vi "PathPlanner_PathFinding_SetGoalPosition.vi"(8 "error in (no error)":errorcluster, 11 "GoalPosition":T1 {"Y" format="%14.3f"; "X" format="%14.3f"}) -> (0 "error out":errorcluster)   [LabVIEW 2019, in "PathPlanner24.lvlib"]
doc: "DOCUMENTATION NOT COMPLETE YET."
uses:
  PathPlanner24.lvlib
  <vilib>/Rock Robotics/WPI/ThirdParty/JAS_Junk/TrajLib/TypeDef/TRANSLATION2D.ctl
  ENum/PathPlanner_PathFinding_Cmd_ENUM.ctl
  <vilib>/Rock Robotics/WPI/ThirdParty/JAS_Junk/TrajLib/Translation2d_GetXY.vi
  PathPlanner_GridPosition_New.vi
  PathPlanner_GridPosition_HashCode.vi
  PathPlanner_PathFinder_GetAllNeighbors.vi
  PathPlanner_GridPosition_Get.vi
  PathPlanner_PathFinder_Globals.vi
  <vilib>/Rock Robotics/WPI/ThirdParty/JAS_Junk/TrajLib/Trajectory_Library.lvlib
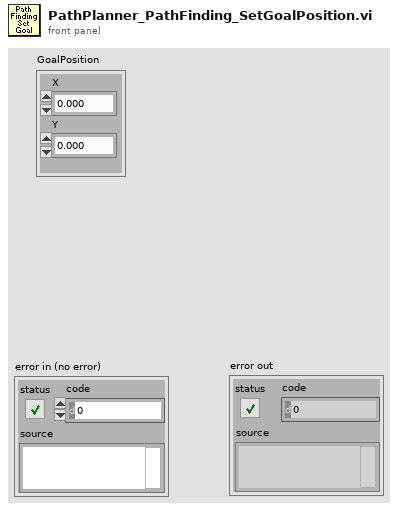
[diagram p1: front panel]
types:
  T1 = typedef "Trajectory_Library.lvlib/TRANSLATION2D.ctl" = cluster{"X":dbl, "Y":dbl}
  T2 = typedef "PathPlanner24.lvlib/PathPlannerFinderGridPosition.ctl" = cluster{"X":i32, "Y":i32}
  T3 = typedef "PathPlanner24.lvlib/PathPlanner_PathFinding_Cmd_ENUM.ctl" = enum16{"Do Nothing", "Reset", "Minor", "Reset and Minor", "Major", "Reset and Major", "Minor and Major", "Reset, Minor, Major"}
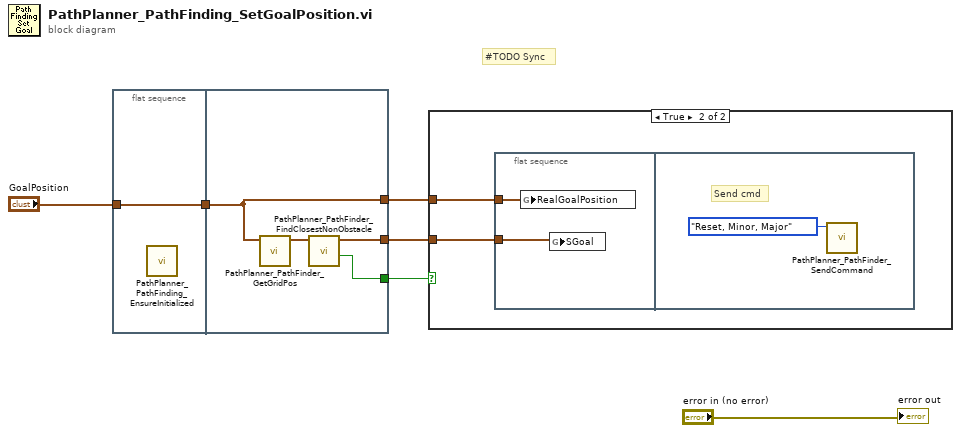
[diagram p0: block diagram]
diagram:
  # "#TODO Sync"
  n1 = flat-sequence {
    tunnel: "GoalPosition" -> [w7]
    tunnel: [w7] -> w2
    tunnel: [w10] -> w6
    tunnel: [w9] -> w5
    tunnel: w2 -> [w8]
    tunnel: [w8] -> w1
    frame #0 {
      n2 = call "PathPlanner_PathFinding_EnsureInitialized.vi"() -> ()  [unwired: 11 in, 1 out]
    }
    frame #1 {
      n3 = call "PathPlanner_PathFinder_GetGridPos.vi"("RealGridPos"=w8) -> ("GridPosition"=w11:T2)  [unwired: 9 in, 1 out]
      n4 = call "PathPlanner_PathFinder_FindClosestNonObstacle.vi"("GridPosition"=w11) -> ("Found"=w10:bool, "NonObstacleGridPositin"=w9:T2)  [unwired: 9 in]
    }
  }
  n5 = case shown="True" w6 {
    tunnel: w5 -> [_ w13]
    tunnel: w1 -> [_ w12]
    frame False {
      # "Not found\nleave alone"
    }
    frame True {
      n6 = flat-sequence {
        tunnel: w13 -> [w15]
        tunnel: w12 -> [w14]
        frame #0 {
          n7 = global write "PathPlanner_PathFinder_Globals.vi" "RealGoalPosition"(w14) -> ()
          n8 = global write "PathPlanner_PathFinder_Globals.vi" "SGoal"(w15) -> ()
        }
        frame #1 {
          # "Send cmd"
          n9 = call "PathPlanner_PathFinder_SendCommand.vi"("PathFindingCommand"=PathPlanner_PathFinding_Cmd_ENUM."Reset, Minor, Major") -> ()  [unwired: 10 in, 1 out]
        }
      }
    }
  }
  "error out" <- "error in (no error)"
